vi "Module Loop.vi"(8 "error in (no error)":errorcluster, 11 "Log Manager Module in":refnum<class "Log Manager Module.lvclass">) -> (0 "error out":errorcluster, 3 "Log Manager Module out":refnum<class "Log Manager Module.lvclass">)   [LabVIEW 2023, in "VolatusData.lvlib" / "Log Manager Module.lvclass"]
uses:
  Log Manager Module.lvclass
  Volatus/Module/Module.lvclass
  Log Preparer Module/Log Preparer Module.lvclass
  Log Manager Module.lvclass/Log Manager Module.ctl
  lv-cdm/CDM-Config/ISO8601 Config.ctl
  lv-cdm/CDM-Config/Format.ctl
  lv-cdm/CDM-Config/Precision.ctl
  lv-cdm/CDM-Config/Timezone.ctl
  messages/StartLog/Data.ctl
  lv-vecto/Vecto/proto/TcpPayload/Data.ctl
  Volatus/Module/Module.lvclass/Module.ctl
  Volatus/MessageQ/MessageQ.lvclass/MessageQ.ctl
  Volatus/StringValue/StringValue.lvclass/StringValue.ctl
  Register Logger.ctl
  Volatus/MessageQ/MessageQ.lvclass
  messages/StartLog/Class/Msg.lvclass
  messages/StartLog/Class/Msg.lvclass/Msg.ctl
  Logger Ready.ctl
  messages/StopLog/Class/Msg.lvclass
  messages/StopLog/Class/Msg.lvclass/Msg.ctl
  messages/StopLog/Data.ctl
  Logger Started.ctl
  Logger Stopped.ctl
  Unregister Logger.ctl
  Volatus/Module/Self Q.vi
  Volatus/MessageQ/Send.vi
  lv-cdm/CDM-Config/ISO-8601 Format Strings.vi
  lv-promises/Promises/Promise/Promise.lvclass
  Volatus/StringValue/StringValue.lvclass
  VolatusData.lvlib
  lv-cdm/CDM-Config/CDM-Config.lvlib
  messages/StartLog/StartLog.lvlib
  lv-vecto/Vecto/proto/TcpPayload/TcpPayload.lvlib
  Log Status Value/Log Status Value.lvclass
  messages/StopLog/StopLog.lvlib
panel:
  in  "Log Series":string
  in  "Log":bool
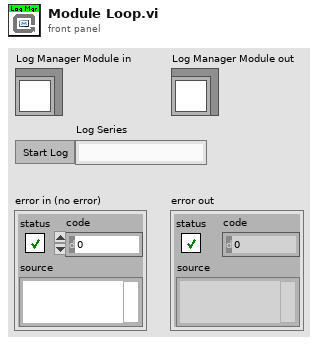
[diagram p1: front panel]
types:
  T1 = enum32{"Invalid", "Standard", "Closed", "Hidden", "Minimized", "Maximized"}
  T2 = typedef "TcpPayload.lvlib/Data.ctl" = cluster{"target_node":u32, "source_id":u32, "sequence":u32, "timestamp":i64, "type":string, "task_id":string, "payload":u8[]}
  T3 = typedef "StartLog.lvlib/Data.ctl" = cluster{"series":string, "timestamp":string, "started_by":string, "groups":string[]}
  T4 = typedef "CDM-Config.lvlib/ISO8601 Config.ctl" = cluster{"Format":T5, "Precision":T6, "Timezone":T7}
  T5 = typedef "CDM-Config.lvlib/Format.ctl" = enum16{"Extended", "Basic"}
  T6 = typedef "CDM-Config.lvlib/Precision.ctl" = enum16{"Millisecond", "Second", "Minute", "Hour", "Day"}
  T7 = typedef "CDM-Config.lvlib/Timezone.ctl" = enum16{"UTC", "Local"}
  T8 = typedef "VolatusData.lvlib/Register Logger.ctl" = cluster{"MsgQ":refnum<class "MessageQ.lvclass">, "ID":string, "Group":string}
  T9 = typedef "VolatusData.lvlib/Logger Ready.ctl" = cluster{"ID":string}
  T10 = typedef "StopLog.lvlib/Data.ctl" = cluster{"reason":string, "groups":string[]}
  T11 = typedef "VolatusData.lvlib/Logger Started.ctl" = cluster{"ID":string}
  T12 = typedef "VolatusData.lvlib/Logger Stopped.ctl" = cluster{"ID":string}
  T13 = typedef "VolatusData.lvlib/Unregister Logger.ctl" = cluster{"ID":string}
  T14 = typedef "VolatusData.lvlib/Log Manager Module.lvclass/Prep Info.ctl" = cluster{"State":T15, "Error":errorcluster}
  T15 = typedef "VolatusData.lvlib/Prep State.ctl" = enum16{"Unknown", "In Progress", "Success", "Failed"}
  T16 = typedef "VolatusData.lvlib/Log Status.ctl" = cluster{"State":T17, "Log":string, "Groups":T18[]}
  T17 = typedef "VolatusData.lvlib/Logging State.ctl" = enum16{"Idle", "Starting", "Logging", "Stopping"}
  T18 = typedef "VolatusData.lvlib/Group State.ctl" = cluster{"Group":string, "State":T19}
  T19 = typedef "VolatusData.lvlib/Logger State.ctl" = enum16{"Unknown", "Idle", "Preparing", "Ready", "Logging", "Stopping"}
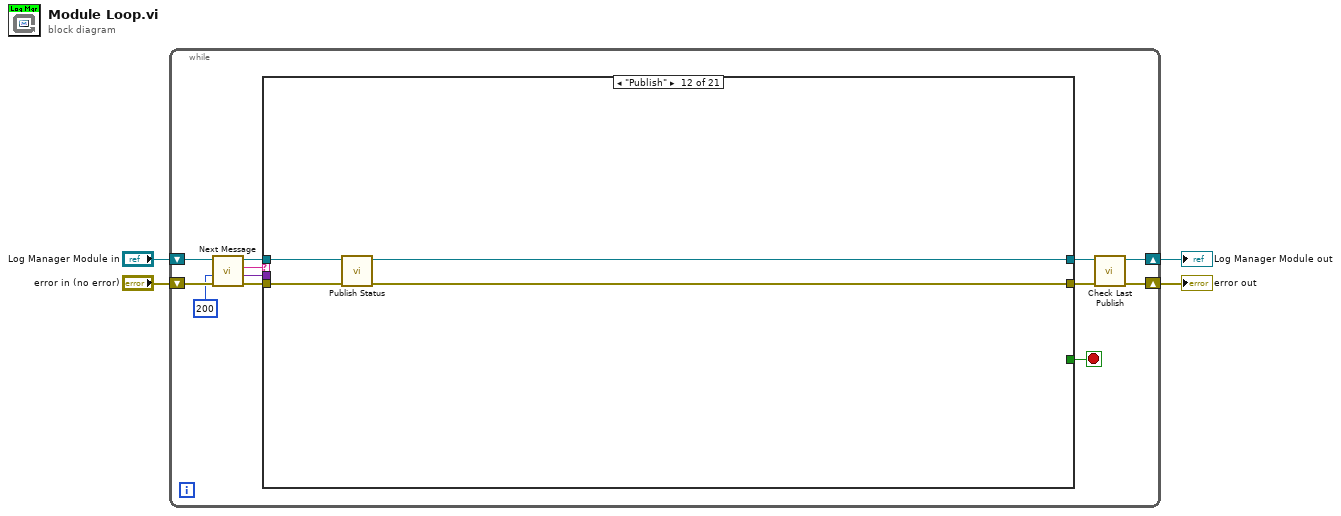
[diagram p0: block diagram]
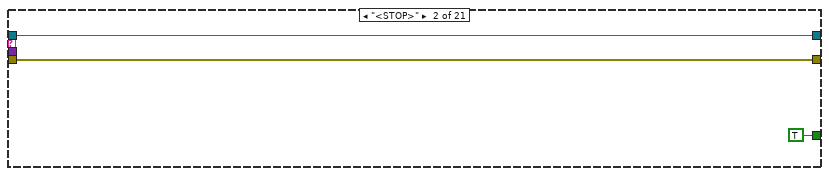
[diagram p3: hidden frame]
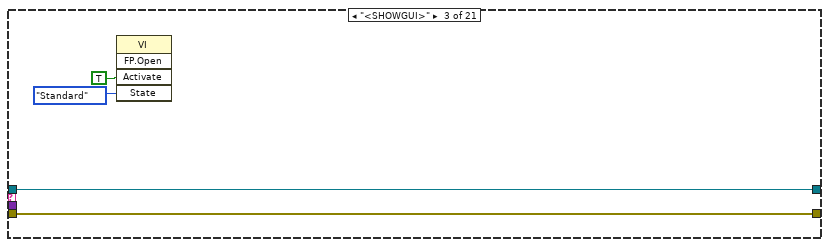
[diagram p4: hidden frame]
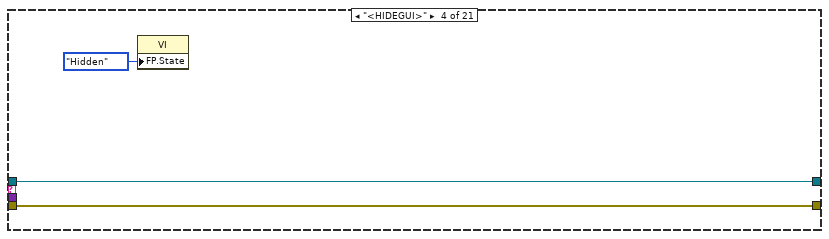
[diagram p5: hidden frame]
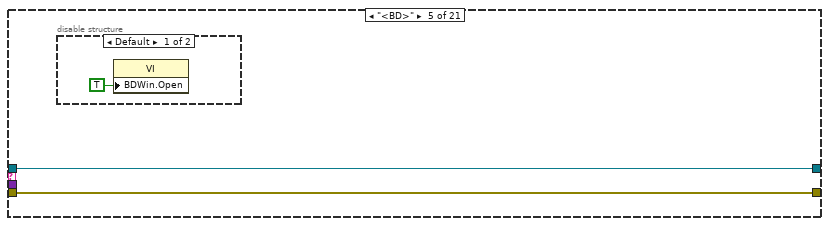
[diagram p6: hidden frame]
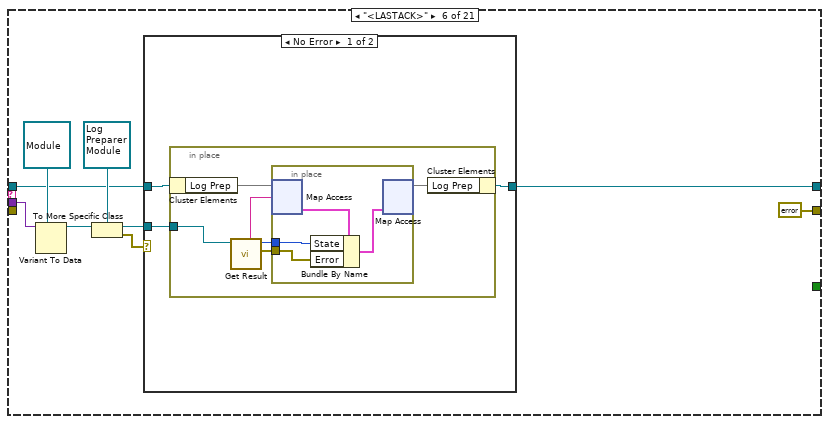
[diagram p8: hidden frame]
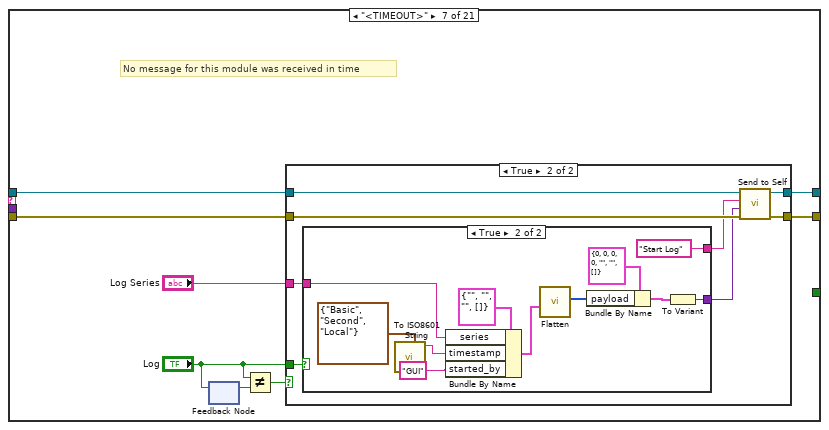
[diagram p10: hidden frame]
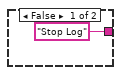
[diagram p12: hidden frame]
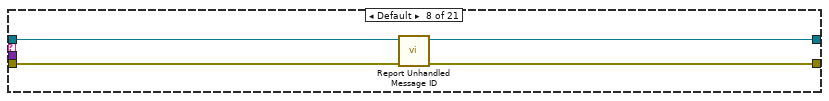
[diagram p13: hidden frame]
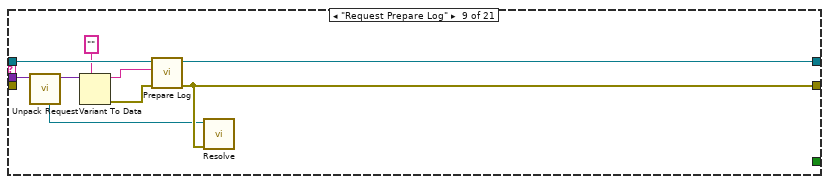
[diagram p14: hidden frame]
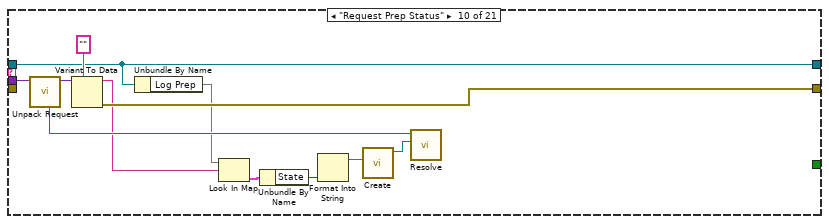
[diagram p15: hidden frame]
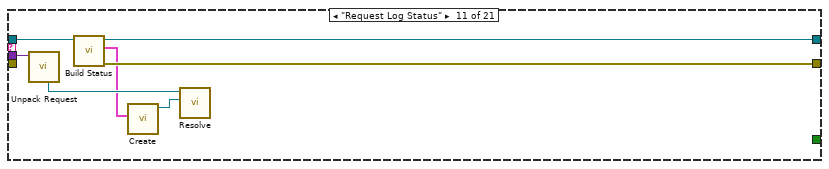
[diagram p16: hidden frame]
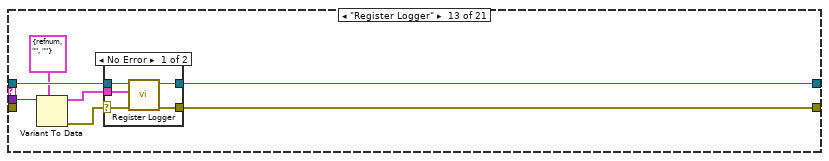
[diagram p17: hidden frame]
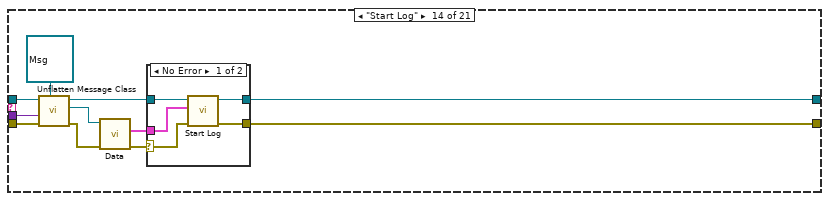
[diagram p19: hidden frame]
diagram:
  n1 = while {
    shift-right: [w5] -> w2
    shift-left: "Log Manager Module in" -> [w16]
    shift-right: [w7] -> w1
    shift-left: "error in (no error)" -> [w15]
    stop <- w11 stop-if-true
    n2 = call "Next Message.vi"("error in (no error)"=w15, "Timeout ms (-1)"=200, "Module in"=w16) -> ("error out"=w14:errorcluster, "Data"=w10:variant, "ID"=w13:string, "Module out"=w12:refnum<class "Log Manager Module.lvclass">)  [unwired: 5 in]
    n3 = case shown="\"Publish\"" w13 {
      tunnel: w14 -> [w17 w20 w24 w27 w29 _ w62 w88 _ _ _ w119 _ w145 _ _ w198 _ _ _ _]
      tunnel: w12 -> [w18 w21 w25 w28 w30 w34 w61 w86 w96 w104 w115 w120 w127 w144 w156 w168 w197 w203 w214 w224 w240]
      tunnel: [w18 w21 w25 w28 w30 w33 w56 w85 w94 w104 w111 w117 w124 w135 w160 w165 w199 w208 w210 w221 w237] -> w6
      tunnel: [_ TRUE _ _ _ _ _ _ _ _ _ _ _ _ _ _ _ _ _ _ _] -> w11
      tunnel: w10 -> [_ _ _ _ _ w40 _ _ w91 w107 w114 _ w126 w143 w159 w167 w190 w207 w217 w223 w239]
      tunnel: [w17 w20 w24 w27 w29 errorcluster {"status"=FALSE, "code"=0, "source"=""} ("error IO") w55 w87 w97 w109 w116 w118 w121 w136 w161 w162 w200 w209 w211 w218 w234] -> w8
      frame "<CLOSE>" {
      }
      frame "<STOP>" {
      }
      frame "<SHOWGUI>" {
        n4 = invoke class="VI" method="FP.Open"("Activate"=TRUE ("Activate?"), "State"=T1."Standard") -> ()  [unwired: 3 in, 5 out]
      }
      frame "<HIDEGUI>" {
        n5 = property class="VI"("FP.State"=T1."Hidden" ("Front Panel Window:State")) -> ()  [unwired: 2 in, 2 out]
      }
      frame "<BD>" {
        n6 = disable-structure shown="Default" {
          frame condition #0 (active) {
            n7 = property class="VI"("BDWin.Open"=TRUE ("Block Diagram Window:Open")) -> ()  [unwired: 2 in, 2 out]
          }
          frame condition #1 {
          }
        }
      }
      frame "<LASTACK>" {
        n8 = Variant To Data(type=refnum<class "Module.lvclass"> refnum ("Volatus:Module"), Variant=w40) -> (data=w38:refnum<class "Module.lvclass">)  [unwired: 1 in, 1 out]
        n9 = To More Specific Class(target class=refnum<class "Log Preparer Module.lvclass"> refnum ("VolatusData:Log Preparer Module.lvclass"), reference=w38) -> (specific class reference=w35:refnum<class "Log Preparer Module.lvclass">, error out=w36:errorcluster)  [unwired: 1 in]
        n10 = case shown="No Error" w36 {
          tunnel: w35 -> [w42 _]
          tunnel: w34 -> [w43 w54]
          tunnel: [w41 w54] -> w33
          frame No Error {
            n11 = in-place {
              in-place-border: w42 -> [w49]
              n12 = in-place-cluster #1(w43) -> ("Log Prep"=w46:map{string, T14})
              n13 = call "Get Result.vi"("Log Preparer Module in"=w49) -> ("error out"=w47:errorcluster, "Result"=w48:T15, "Log"=w45:string)  [unwired: 8 in]
              n14 = in-place {
                in-place-border: w48 -> [w52]
                in-place-border: w47 -> [w53]
                n15 = in-place-map #2(w46, w45) -> (w50:T14)  [unwired: 1 in, 1 out]
                n16 = Bundle By Name(cluster=w50, "State"=w52, "Error"=w53) -> (w51:T14)
                n17 = in-place-map #2(w51) -> (w44:map{string, T14})  [unwired: 1 in, 2 out]
              }
              n18 = in-place-cluster #1("Log Prep"=w44) -> (w41:refnum<class "Log Manager Module.lvclass">)
            }
          }
          frame Error {
          }
        }
      }
      frame "<TIMEOUT>" {
        # "No message for this module was received in time"
        n19 = feedback-in #3("Log") -> ()
        n20 = feedback #3() -> (w60:bool)  [unwired: 1 in]
        n21 = Not Equal?(x="Log", y=w60) -> (x != y?=w59:bool)
        n22 = case shown="True" w59 {
          tunnel: w61 -> [w64 w72]
          tunnel: "Log" -> [_ w65]
          tunnel: "Log Series" -> [_ w68]
          tunnel: w62 -> [w63 w71]
          tunnel: [w64 w70] -> w56
          tunnel: [w63 w69] -> w55
          frame False {
          }
          frame True {
            n23 = case shown="True" w65 {
              tunnel: w68 -> [_ w82]
              tunnel: ["Stop Log" ("Message ID") "Start Log" ("Message ID")] -> w67
              tunnel: [_ w78] -> w66
              frame False {
              }
              frame True {
                n24 = call "To ISO8601 String.vi"("Format Config"=T4 {"Format"=enum."Basic", "Precision"=enum."Second", "Timezone"=enum."Local"}) -> ("ISO 8601"=w81:string)  [unwired: 10 in]
                n25 = Bundle By Name(cluster=T3 {"series"="", "timestamp"="", "started_by"="", "groups"=[]} ("StartLog"), "series"=w82, "timestamp"=w81, "started_by"="GUI") -> (w77:T3)
                n26 = call "Flatten.vi"("Data"=w77) -> ("Buffer"=w74:u8[])  [unwired: 9 in, 1 out]
                n27 = Bundle By Name(cluster=T2 {"target_node"=0, "source_id"=0, "sequence"=0, "timestamp"=0, "type"="", "task_id"="", "payload"=[]} ("TcpPayload"), "payload"=w74) -> (w75:T2)
                n28 = To Variant(anything=w75) -> (Variant=w78:variant)
              }
            }
            n29 = call "Send to Self.vi"("error in (no error)"=w71, "Data"=w66, "Message ID"=w67, "Module in"=w72) -> ("error out"=w69:errorcluster, "Module out"=w70:refnum<class "Log Manager Module.lvclass">)  [unwired: 6 in]
          }
        }
      }
      frame Default {
        n30 = call "Report Unhandled Message ID.vi"("error in (no error)"=w88, "Module in"=w86) -> ("error out"=w87:errorcluster, "Module out"=w85:refnum<class "Log Manager Module.lvclass">)  [unwired: 8 in]
      }
      frame "Request Prepare Log" {
        n31 = call "Unpack Request.vi"("Request Data"=w91) -> ("Data"=w90:variant, "Promise"=w89:refnum<class "Promise.lvclass">)  [unwired: 8 in, 1 out]
        n32 = Variant To Data(type="", Variant=w90) -> (data=w93:string, error out=w92:errorcluster)  [unwired: 1 in]
        n33 = call "Prepare Log.vi"("error in (no error)"=w92, "Log"=w93, "Log Manager Module in"=w96) -> ("error out"=w97:errorcluster, "Log Manager Module out"=w94:refnum<class "Log Manager Module.lvclass">)  [unwired: 7 in]
        n34 = call "Resolve.vi"("error in (no error)"=w97, "Promise in"=w89) -> ()  [unwired: 8 in, 2 out]
      }
      frame "Request Prep Status" {
        n35 = call "Unpack Request.vi"("Request Data"=w107) -> ("Data"=w106:variant, "Promise"=w105:refnum<class "Promise.lvclass">)  [unwired: 8 in, 1 out]
        n36 = Variant To Data(type="", Variant=w106) -> (data=w102:string, error out=w109:errorcluster)  [unwired: 1 in]
        n37 = Unbundle By Name(w104) -> ("Log Prep"=w103:map{string, T14})
        n38 = Look In Map(map=w103, key=w102) -> (value=w101:T14)  [unwired: 1 in, 1 out]
        n39 = Unbundle By Name(w101) -> ("State"=w100:T15)
        n40 = Format Into String(w100) -> (resulting string=w99:string)  [unwired: 3 in, 1 out]
        n41 = call "Create.vi"("Value"=w99) -> ("StringValue out"=w98:refnum<class "StringValue.lvclass">)  [unwired: 10 in]
        n42 = call "Resolve.vi"("Result (None)"=w98, "Promise in"=w105) -> ()  [unwired: 8 in, 2 out]
      }
      frame "Request Log Status" {
        n43 = call "Unpack Request.vi"("Request Data"=w114) -> ("Promise"=w113:refnum<class "Promise.lvclass">)  [unwired: 8 in, 2 out]
        n44 = call "Build Status.vi"("Log Manager Module in"=w115) -> ("error out"=w116:errorcluster, "Logging State"=w110:T16, "Log Manager Module out"=w111:refnum<class "Log Manager Module.lvclass">)  [unwired: 8 in]
        n45 = call "Create.vi"("Log Status"=w110) -> ("Log Status Value out"=w112:refnum<class "Log Status Value.lvclass">)  [unwired: 10 in]
        n46 = call "Resolve.vi"("Result (None)"=w112, "Promise in"=w113) -> ()  [unwired: 8 in, 2 out]
      }
      frame "Publish" {
        n47 = call "Publish Status.vi"("error in (no error)"=w119, "Log Manager Module in"=w120) -> ("error out"=w118:errorcluster, "Log Manager Module out"=w117:refnum<class "Log Manager Module.lvclass">)  [unwired: 8 in]
      }
      frame "Register Logger" {
        n48 = Variant To Data(type=T8 {"MsgQ"=refnum, "ID"="", "Group"=""} ("Logger Registration"), Variant=w126) -> (data=w123:T8, error out=w122:errorcluster)  [unwired: 1 in]
        n49 = case shown="No Error" w122 {
          selector: w122 -> [w129 w133]
          tunnel: w127 -> [w132 w134]
          tunnel: [w131 w134] -> w124
          tunnel: w123 -> [w130 _]
          tunnel: [w128 w133] -> w121
          frame No Error {
            n50 = call "Register Logger.vi"("error in (no error)"=w129, "Logger Registration"=w130, "Log Manager Module in"=w132) -> ("error out"=w128:errorcluster, "Log Manager Module out"=w131:refnum<class "Log Manager Module.lvclass">)  [unwired: 7 in]
          }
          frame Error {
          }
        }
      }
      frame "Start Log" {
        n51 = call "Unflatten Message Class.vi"("Message Type"=refnum<class "Msg.lvclass"> refnum ("StartLog.lvlib:Msg.lvclass"), "error in (no error)"=w145, "Data"=w143, "Module in"=w144) -> ("error out"=w141:errorcluster, "Message"=w140:refnum<class "Msg.lvclass">, "Module out"=w137:refnum<class "Log Manager Module.lvclass">)  [unwired: 4 in, 1 out]
        n52 = call "Data.vi"("error in (no error)"=w141, "PB Msg Template in"=w140) -> ("error out"=w139:errorcluster, "Data"=w138:T3)  [unwired: 7 in, 1 out]
        n53 = case shown="No Error" w139 {
          selector: w139 -> [w148 w151]
          tunnel: w138 -> [w149 _]
          tunnel: w137 -> [w150 w152]
          tunnel: [w147 w151] -> w136
          tunnel: [w146 w152] -> w135
          frame No Error {
            n54 = call "Start Log.vi"("error in (no error)"=w148, "Data"=w149, "Log Manager Module in"=w150) -> ("error out"=w147:errorcluster, "Log Manager Module out"=w146:refnum<class "Log Manager Module.lvclass">)  [unwired: 7 in]
          }
          frame Error {
          }
        }
      }
      frame "Request Start Log" {
        n55 = call "Unpack Request.vi"("Request Data"=w159) -> ("Data"=w158:variant, "Promise"=w153:refnum<class "Promise.lvclass">)  [unwired: 8 in, 1 out]
        n56 = Variant To Data(type=T3 {"series"="", "timestamp"="", "started_by"="", "groups"=[]} ("Data"), Variant=w158) -> (data=w155:T3, error out=w154:errorcluster)  [unwired: 1 in]
        n57 = call "Start Log.vi"("error in (no error)"=w154, "Data"=w155, "Log Manager Module in"=w156) -> ("error out"=w161:errorcluster, "Log Manager Module out"=w160:refnum<class "Log Manager Module.lvclass">)  [unwired: 7 in]
        n58 = call "Resolve.vi"("error in (no error)"=w161, "Promise in"=w153) -> ()  [unwired: 8 in, 2 out]
      }
      frame "Logger Ready" {
        n59 = Variant To Data(type=T9 {"ID"=""} ("Logger Ready"), Variant=w167) -> (data=w163:T9, error out=w164:errorcluster)  [unwired: 1 in]
        n60 = case shown="No Error" w164 {
          selector: w164 -> [w174 w188]
          tunnel: w168 -> [w170 w189]
          tunnel: [w171 w189] -> w165
          tunnel: w163 -> [w173 _]
          tunnel: [w172 w188] -> w162
          frame No Error {
            n61 = Unbundle By Name(w170) -> ("State"=w169:T17)
            n62 = case shown="\"Starting\"" w169 {
              selector: w169 -> [w177 _]
              tunnel: w174 -> [_ w187]
              tunnel: w173 -> [_ w186]
              tunnel: [w175 w184] -> w172
              tunnel: [w180 w182] -> w171
              tunnel: w170 -> [w180 w181]
              frame Default {
                n63 = Format Into String(format string="Must be in Starting state to update logger readiness, instead in \"%s\" state.", w177) -> (resulting string=w176:string)  [unwired: 2 in, 1 out]
                n64 = call <vilib>:"Error Cluster From Error Code.vi"("error message (\"\")"=w176, "error code (0)"=-909) -> ("error out"=w175:errorcluster)  [unwired: 7 in]
              }
              frame "Starting" {
                n65 = call "Logger Ready.vi"("error in (no error)"=w187, "Logger Ready"=w186, "Log Manager Module in"=w181) -> ("error out"=w185:errorcluster, "Log Manager Module out"=w183:refnum<class "Log Manager Module.lvclass">)  [unwired: 7 in]
                n66 = call "Start If All Ready.vi"("error in (no error)"=w185, "Log Manager Module in"=w183) -> ("error out"=w184:errorcluster, "Log Manager Module out"=w182:refnum<class "Log Manager Module.lvclass">)  [unwired: 8 in]
              }
            }
          }
          frame Error {
          }
        }
      }
      frame "Stop Log" {
        n67 = call "Unflatten Message Class.vi"("Message Type"=refnum<class "Msg.lvclass"> refnum ("StopLog.lvlib:Msg.lvclass"), "error in (no error)"=w198, "Data"=w190, "Module in"=w197) -> ("error out"=w193:errorcluster, "Message"=w194:refnum<class "Msg.lvclass">, "Module out"=w196:refnum<class "Log Manager Module.lvclass">)  [unwired: 4 in, 1 out]
        n68 = call "Data.vi"("error in (no error)"=w193, "PB Msg Template in"=w194) -> ("error out"=w191:errorcluster, "Data"=w192:T10)  [unwired: 7 in, 1 out]
        n69 = call "Stop Log.vi"("error in (no error)"=w191, "Data"=w192, "Log Manager Module in"=w196) -> ("error out"=w200:errorcluster, "Log Manager Module out"=w199:refnum<class "Log Manager Module.lvclass">)  [unwired: 7 in]
      }
      frame "Request Stop Log" {
        n70 = call "Unpack Request.vi"("Request Data"=w207) -> ("Data"=w206:variant, "Promise"=w202:refnum<class "Promise.lvclass">)  [unwired: 8 in, 1 out]
        n71 = Variant To Data(type=T10 {"reason"="", "groups"=[]} ("Data"), Variant=w206) -> (data=w204:T10, error out=w201:errorcluster)  [unwired: 1 in]
        n72 = call "Stop Log.vi"("error in (no error)"=w201, "Data"=w204, "Log Manager Module in"=w203) -> ("error out"=w209:errorcluster, "Log Manager Module out"=w208:refnum<class "Log Manager Module.lvclass">)  [unwired: 7 in]
        n73 = call "Resolve.vi"("error in (no error)"=w209, "Promise in"=w202) -> ()  [unwired: 8 in, 2 out]
      }
      frame "Logger Started" {
        n74 = Variant To Data(type=T11 {"ID"=""} ("Logger Started"), Variant=w217) -> (data=w215:T11, error out=w212:errorcluster)  [unwired: 1 in]
        n75 = Unbundle By Name(w215) -> ("ID"=w213:string)
        n76 = call "Logger Started.vi"("error in (no error)"=w212, "ID"=w213, "Log Manager Module in"=w214) -> ("error out"=w211:errorcluster, "Log Manager Module out"=w210:refnum<class "Log Manager Module.lvclass">)  [unwired: 7 in]
      }
      frame "Logger Stopped" {
        n77 = Variant To Data(type=T12 {"ID"=""} ("Logger Stopped"), Variant=w223) -> (data=w219:T12, error out=w220:errorcluster)  [unwired: 1 in]
        n78 = case shown="No Error" w220 {
          selector: w220 -> [w229 w232]
          tunnel: w224 -> [w231 w233]
          tunnel: [w227 w233] -> w221
          tunnel: w219 -> [w228 _]
          tunnel: [w225 w232] -> w218
          frame No Error {
            n79 = call "Logger Stopped.vi"("error in (no error)"=w229, "Logger Stopped"=w228, "Log Manager Module in"=w231) -> ("error out"=w226:errorcluster, "Log Manager Module out"=w230:refnum<class "Log Manager Module.lvclass">)  [unwired: 7 in]
            n80 = call "Check All Stopped.vi"("error in (no error)"=w226, "Log Manager Module in"=w230) -> ("error out"=w225:errorcluster, "Log Manager Module out"=w227:refnum<class "Log Manager Module.lvclass">)  [unwired: 7 in, 1 out]
          }
          frame Error {
          }
        }
      }
      frame "Unregister Logger" {
        n81 = Variant To Data(type=T13 {"ID"=""} ("Unregister Logger"), Variant=w239) -> (data=w235:T13, error out=w236:errorcluster)  [unwired: 1 in]
        n82 = case shown="No Error" w236 {
          selector: w236 -> [w243 w246]
          tunnel: w240 -> [w245 w247]
          tunnel: [w244 w247] -> w237
          tunnel: w235 -> [w242 _]
          tunnel: [w241 w246] -> w234
          frame No Error {
            n83 = call "Unregister Logger.vi"("error in (no error)"=w243, "Unregister Logger"=w242, "Log Manager Module in"=w245) -> ("error out"=w241:errorcluster, "Log Manager Module out"=w244:refnum<class "Log Manager Module.lvclass">)  [unwired: 7 in]
          }
          frame Error {
          }
        }
      }
    }
    n84 = call "Check Last Publish.vi"("error in (no error)"=w8, "Log Manager Module in"=w6) -> ("error out"=w7:errorcluster, "Log Manager Module out"=w5:refnum<class "Log Manager Module.lvclass">)  [unwired: 8 in]
  }
  "error out" <- w1
  "Log Manager Module out" <- w2
